vi "Init.vi"(7 "I2C #":T2=-1, 8 "error in (no error)":errorcluster, 9 "Address":T1=37 format="%02x", 10 "Session In":refnum<class "Session.lvclass">) -> (0 "error out":errorcluster, 3 "M5Stack8ChPWM Out":refnum<class "M5Stack I2C 8Ch Servo.lvclass">)   [LabVIEW 2020, in "CTI-Peripheral.lvlib" / "M5Stack I2C 8Ch Servo.lvclass"]
uses:
  M5Stack I2C 8Ch Servo.lvclass
  CTI/Session/Session.lvclass
  CTI/I2C Number.ctl
  CTI/I2C Address.ctl
  CTI/I2C Connection/I2C Connection.lvclass/I2C Connection.ctl
  M5Stack I2C 8Ch Servo.lvclass/M5Stack I2C 8Ch Servo.ctl
  CTI/I2C Connection/I2C Connection.lvclass
  CTI/CTI.lvlib
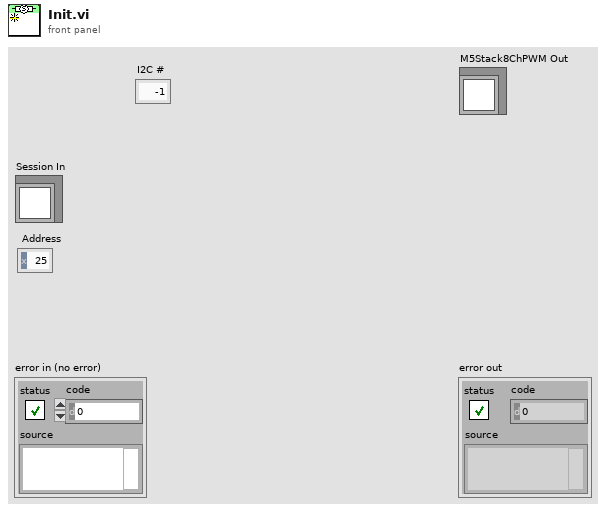
[diagram p1: front panel]
types:
  T1 = typedef "CTI.lvlib/I2C Address.ctl" = u8
  T2 = typedef "CTI.lvlib/I2C Number.ctl" = i8
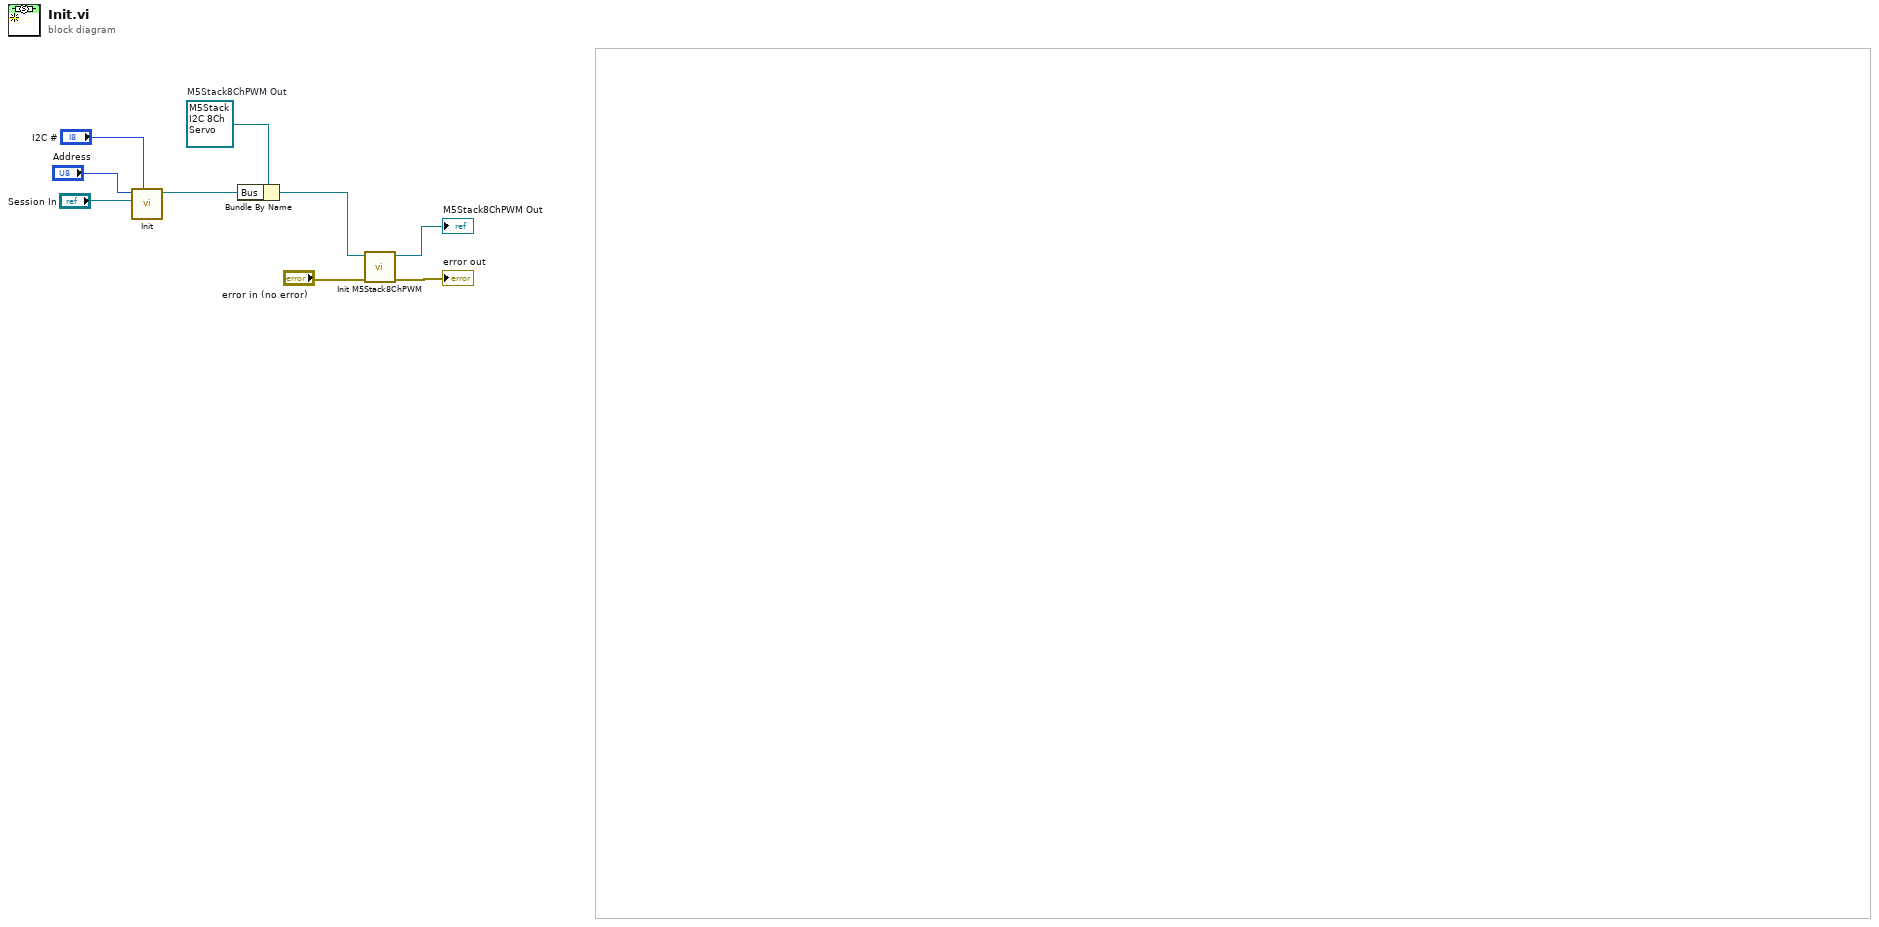
[diagram p0: block diagram]
diagram:
  w1 = refnum<class "M5Stack I2C 8Ch Servo.lvclass"> refnum  # M5Stack8ChPWM Out
  n1 = call "Init.vi"("I2C #"="I2C #", "Session"="Session In", "Address"="Address") -> ("I2C Connection"=w9:refnum<class "I2C Connection.lvclass">)  [unwired: 7 in, 1 out]
  n2 = Bundle By Name(cluster=w1, "Bus"=w9) -> (w3:refnum<class "M5Stack I2C 8Ch Servo.lvclass">)
  n3 = call "Init M5Stack8ChPWM.vi"("error in (no error)"="error in (no error)", "M5Stack I2C 8Ch Servo in"=w3) -> ("error out"=→"error out":errorcluster, "M5Stack I2C 8Ch Servo out"=→"M5Stack8ChPWM Out":refnum<class "M5Stack I2C 8Ch Servo.lvclass">)  [unwired: 8 in]
